vi "get_table.vi"(8 "error in (no error)":errorcluster, 10 "table_name":string, 11 "Doc in":refnum<class "Doc.lvclass">) -> (0 "error out":errorcluster, 1 "Table":refnum<class "Table.lvclass">, 2 "found?":bool, 3 "Doc out":refnum<class "Doc.lvclass">)   [LabVIEW 2020, in "toml_edit.lvlib" / "Doc.lvclass"]
uses:
  Doc.lvclass
  Table/Table.lvclass
  Doc.lvclass/Doc.ctl
  dragon_toml_64.dll
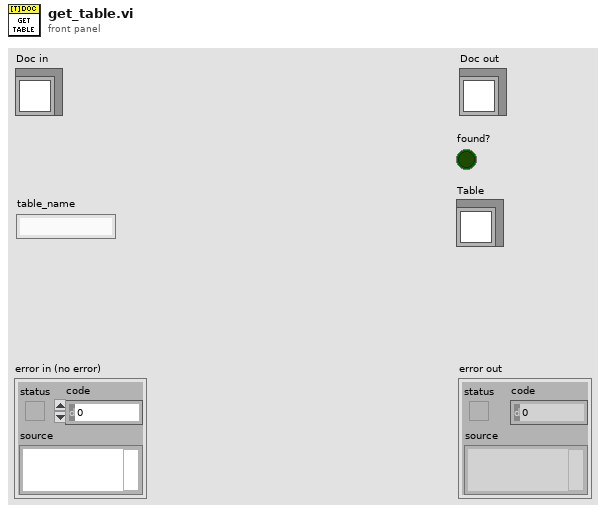
[diagram p1: front panel]
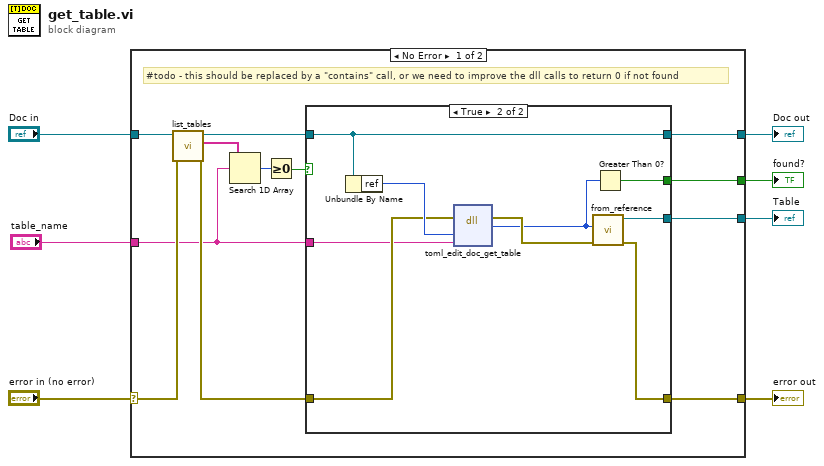
[diagram p0: block diagram]
diagram:
  n1 = case shown="No Error" "error in (no error)" {
    selector: "error in (no error)" -> [w15 w32]
    tunnel: [w18 w32] -> w6
    tunnel: [w9 w31] -> w4
    tunnel: "Doc in" -> [w16 w31]
    tunnel: "table_name" -> [w12 _]
    tunnel: [w19 _] -> w2
    tunnel: [w8 _] -> w1
    frame No Error {
      # "#todo - this should be replaced by a \"contains\" call, or we need to improve the dll calls to return 0 if not found"
      n2 = call "list_tables.vi"("error in (no error)"=w15, "Doc in"=w16) -> ("error out"=w14:errorcluster, "table_names"=w13:string[], "Doc out"=w17:refnum<class "Doc.lvclass">)  [unwired: 7 in]
      n3 = Search 1D Array(1D array=w13, element=w12) -> (index of element=w11:i32)  [unwired: 1 in]
      n4 = Greater Or Equal To 0?(x=w11) -> (x >= 0?=w10:bool)
      n5 = case shown="True" w10 {
        tunnel: [_ w28] -> w19
        tunnel: [w20 w27] -> w18
        tunnel: w17 -> [w21 w24]
        tunnel: w14 -> [w20 w26]
        tunnel: w12 -> [_ w25]
        tunnel: [w21 w24] -> w9
        tunnel: [_ w22] -> w8
        frame False {
        }
        frame True {
          n6 = Unbundle By Name(w24) -> ("ref"=w30:u64)
          n7 = dll-call lib="C:/projects/dragon-desktop/source/submodules/toml-edit-labview/lv_src/dragon_toml_*.dll" fn="toml_edit_doc_get_table"(error in=w26, "doc_ref"=w30, "table_name"=w25) -> (error out=w29:errorcluster, "table_ptr"=w23:u64)  [unwired: 4 in, 1 out]
          n8 = call "from_reference.vi"("error in (no error)"=w29, "ref"=w23) -> ("error out"=w27:errorcluster, "Table out"=w28:refnum<class "Table.lvclass">)  [unwired: 8 in]
          n9 = Greater Than 0?(x=w23) -> (x > 0?=w22:bool)
        }
      }
    }
    frame Error {
    }
  }
  "error out" <- w6
  "Doc out" <- w4
  "Table" <- w2
  "found?" <- w1
